vi "VIH Constant - ProjFile - Root Tag Name.vi"() -> (3 "Tag Name":string)   [LabVIEW 2014]
doc: "::: VI Helpeks :::\nCopyright (c) 2000-2026 Konstantin Shifershteyn. All rights reserved."
panel:
  # "VI Helpeks\nCopyright (c) 2012-2026 Konstantin Shifershteyn"
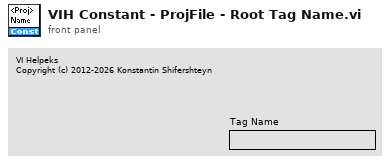
[diagram p1: front panel]
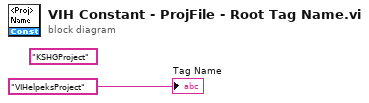
[diagram p0: block diagram]
diagram:
  (unwired) "KSHGProject" ("Tag Name")
  "Tag Name" <- "VIHelpeksProject" ("Tag Name")
